vi "Host_Publish_Config.vi"(8 "error in (no error)":errorcluster={"status"=FALSE, "code"=0, "source"="\"\""}, 10 "version":string, 11 "Validated config":string) -> (0 "error out":errorcluster={"status"=FALSE, "code"=0, "source"="\"\""}, 2 "status ok":bool, 3 "Publish receipt":string)   [LabVIEW 2026]
doc: "INTENT: Publish a fixed configuration revision. LOGIC: Serialize signed/hashed revision as approved by project policy; transfer, await target validation and acknowledgement."
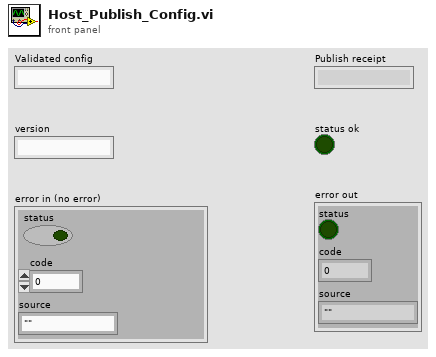
[diagram p1: front panel]
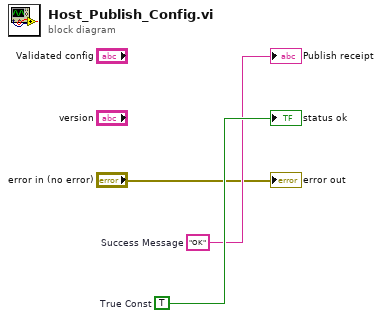
[diagram p0: block diagram]
diagram:
  w3 = TRUE  # True Const
  w2 = "OK"  # Success Message
  "Publish receipt" <- w2
  "status ok" <- w3
  "error out" <- "error in (no error)"
